vi "Two Way Event Recorder GUID Lookup.vi"() -> ()   [LabVIEW 2015, in "Two Way Event Recorder Custom Device.lvlib"]
doc: "Use this Global VI to access the GUIDs assigned to the page resources of the Custom Device."
uses:
  Two Way Event Recorder Custom Device.lvlib
panel:
  in  "Custom Device":string="1624b228-eb50-414f-b33d-05f9457d2721"
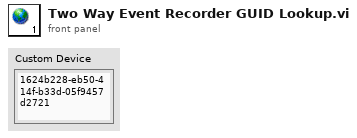
[diagram p1: front panel]
diagram:
